vi "Update Children.vi"(6 "Labels":map{string, string}(c390), 8 "error in (no error)":errorcluster, 9 "Created?":bool=TRUE, 10 "New Value":dbl, 11 "Histogram in":refnum<class "Histogram.lvclass">) -> (0 "error out":errorcluster, 3 "Histogram out":refnum<class "Histogram.lvclass">)   [LabVIEW 2020, in "Metrics.lvlib" / "Histogram.lvclass"]
uses:
  Histogram.lvclass
  sample/Edit Action.ctl
  Histogram.lvclass/Histogram.ctl
  metric/Metric.lvclass
  sample/Sample.lvclass
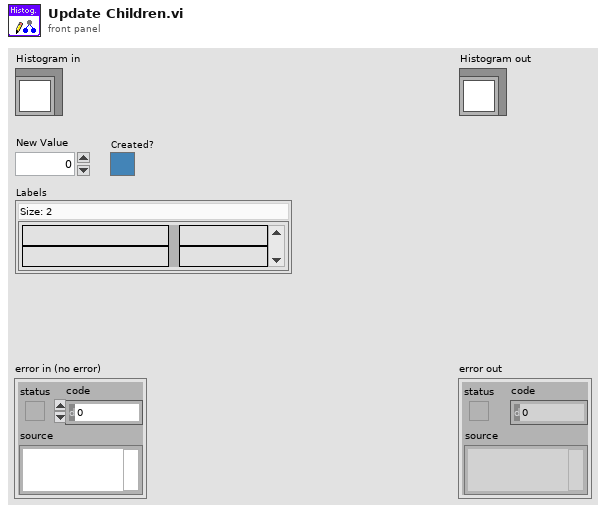
[diagram p1: front panel]
types:
  T1 = typedef "Metrics.lvlib/Sample.lvclass/Edit Action.ctl" = enum16{"Set", "Increment"}
  T2 = enum16{"seconds", "milliseconds", "microseconds"}
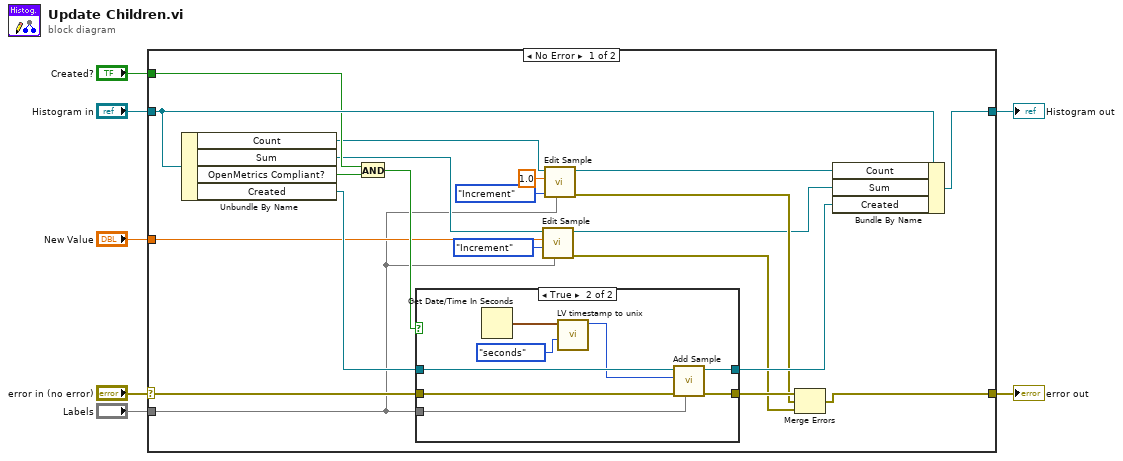
[diagram p0: block diagram]
diagram:
  n1 = case shown="No Error" "error in (no error)" {
    selector: "error in (no error)" -> [w25 w40]
    tunnel: [w9 w40] -> w6
    tunnel: [w13 w39] -> w4
    tunnel: "Histogram in" -> [w26 w39]
    tunnel: "Labels" -> [w14 _]
    tunnel: "Created?" -> [w24 _]
    tunnel: "New Value" -> [w16 _]
    frame No Error {
      n2 = Unbundle By Name(w26) -> ("Count"=w21:refnum<class "Metric.lvclass">, "Sum"=w17:refnum<class "Metric.lvclass">, "OpenMetrics Compliant?"=w23:bool, "Created"=w27:refnum<class "Metric.lvclass">)
      n3 = And(x=w24, y=w23) -> (x .and. y?=w22:bool)
      n4 = case shown="True" w22 {
        tunnel: w27 -> [w30 w38]
        tunnel: w14 -> [_ w34]
        tunnel: [w30 w33] -> w28
        tunnel: w25 -> [w29 w31]
        tunnel: [w29 w32] -> w12
        frame False {
        }
        frame True {
          n5 = Get Date/Time In Seconds() -> (seconds since 1Jan1904=w37:timestamp)
          n6 = call "LV timestamp to unix.vi"("Precision (ms)"=T2."seconds", "Timestamp"=w37) -> ("Unix epoch time"=w35:u64)  [unwired: 9 in]
          n7 = call-dynamic "Add Sample.vi"("Labels"=w34, "error in (no error)"=w31, "Value"=w35, "Metric in"=w38) -> ("error out"=w32:errorcluster, "Metric out"=w33:refnum<class "Metric.lvclass">)  [unwired: 6 in]
        }
      }
      n8 = call "Edit Sample.vi"("Labels"=w14, "Action"=Edit_Action."Increment", "Step"=w16, "Metric in"=w17) -> ("error out"=w10:errorcluster, "Metric out"=w8:refnum<class "Metric.lvclass">)  [unwired: 5 in, 1 out]
      n9 = call "Edit Sample.vi"("Labels"=w14, "Action"=Edit_Action."Increment", "Step"=1.0, "Metric in"=w21) -> ("error out"=w11:errorcluster, "Metric out"=w18:refnum<class "Metric.lvclass">)  [unwired: 5 in, 1 out]
      n10 = Merge Errors(w12, w11, w10) -> (w9:errorcluster)
      n11 = Bundle By Name(cluster=w26, "Count"=w18, "Sum"=w8, "Created"=w28) -> (w13:refnum<class "Histogram.lvclass">)
    }
    frame Error {
    }
  }
  "error out" <- w6
  "Histogram out" <- w4
